vi "create available tags menu.vi"(5 "reference":refnum<vi>, 7 "channel action event":refnum<user-event>, 8 "error in":errorcluster, 9 "channel to map to":refnum<class "TBM channel.lvclass">, 10 "Coords":T1, 11 "engine configuration in":refnum<class "engine configuration.lvclass">) -> (0 "error out":errorcluster)   [LabVIEW 2013, in "control module editor.lvclass"]
uses:
  control module editor.lvclass
  <vilib>/NI/Module Execution Interface/Engine Configuration/engine configuration.lvclass
  <vilib>/NI/Tag Bus Module Framework/channel/TBM channel.lvclass
  Table API/Available Tag Menu/channel action event.ctl
  Table API/Available Tag Menu/dialog output action.ctl
  <vilib>/NI/Tag Bus/tag/tag descriptor.lvclass
  Table API/Table Manager/Call Back Ref Type Def.ctl
  Configuration Editor/Classes/Engine Parent/Engine Parent Editor Node.lvclass
  Configuration Editor/Classes/Module editor node/module editor node.lvclass
  <vilib>/Utility/miscctls.llb/LVPoint32TypeDef.ctl
  tag select dialog.vi
  Table API/Table Manager.lvlib
  Table API/Table Manager/Table Manager.lvclass
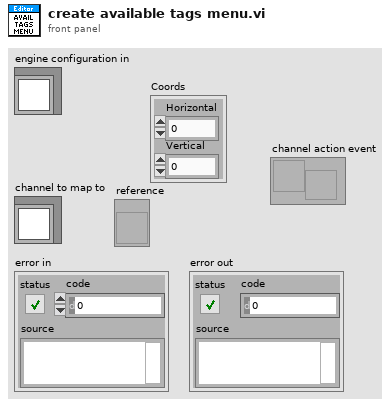
[diagram p1: front panel]
types:
  T1 = typedef "LVPoint32TypeDef.ctl" = cluster{"Horizontal":i32, "Vertical":i32}
  T2 = enum32{"Invalid", "Standard", "Closed", "Hidden", "Minimized", "Maximized"}
  T3 = typedef "LVRectTypeDef.ctl" = cluster{"Left":i16, "Top":i16, "Right":i16, "Bottom":i16}
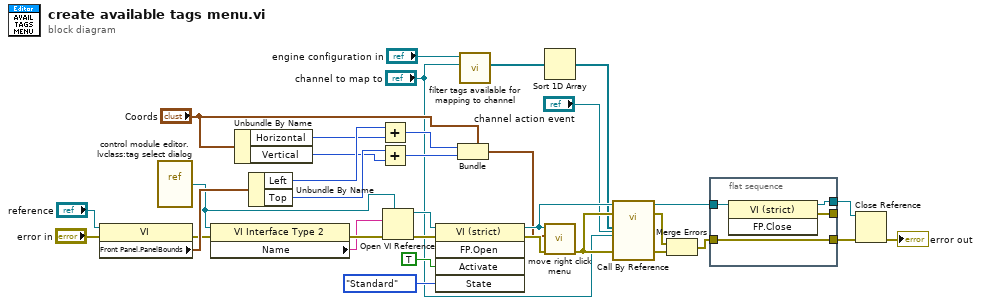
[diagram p0: block diagram]
diagram:
  n1 = property class="VI"(reference="reference", error in="error in") -> (error out=w9:errorcluster, "Front Panel.PanelBounds"=w32:T3)  [unwired: 1 out]
  n2 = vi-ref "control module editor.lvclass:tag select dialog.vi"() -> (w16:refnum<vi>)
  n3 = property class="VI Interface Type 2"(reference=w16, error in=w9) -> (error out=w23:errorcluster, "Name"=w22:string)  [unwired: 1 out]
  n4 = Unbundle By Name("Coords") -> ("Horizontal"=w30:i32, "Vertical"=w27:i32)
  n5 = Unbundle By Name(w32) -> ("Left"=w31:i16, "Top"=w28:i16)
  n6 = Add(x=w31, y=w30) -> (x+y=w29:i32)
  n7 = Add(x=w28, y=w27) -> (x+y=w26:i32)
  n8 = Open VI Reference(type specifier VI Refnum (for type only)=w16, vi path=w22, error in (no error)=w23) -> (vi reference=w20:refnum<vi>, error out=w21:errorcluster)  [unwired: 3 in]
  n9 = invoke class="VI (strict)" method="FP.Open"(reference=w20, error in=w21, "Activate"=TRUE ("Activate?"), "State"=T2."Standard") -> (reference out=w15:refnum<vi>, error out=w17:errorcluster)  [unwired: 1 in, 3 out]
  n10 = Bundle(cluster="Coords", "Horizontal"=w29, "Vertical"=w26) -> (w3:T1)
  n11 = call <vilib>:"filter tags available for mapping to channel.vi"("channel to map to"="channel to map to", "engine configuration in"="engine configuration in") -> ("filtered tags"=w33:refnum<class "tag descriptor.lvclass">[])  [unwired: 8 in, 1 out]
  n12 = Sort 1D Array(array=w33) -> (sorted array=w5:refnum<class "tag descriptor.lvclass">[])
  n13 = call "move right click menu.vi"("error in"=w17, "Point32"=w3, "VI"=w15) -> ("error out"=w7:errorcluster)  [unwired: 8 in]
  n14 = call-by-ref "?"(reference=w15, error in=w7, "channel action event"="channel action event", "error in"=w7, "channel to map to"="channel to map to", "filtered tags"=w5) -> (reference out=w13:refnum<vi>, error out=w14:errorcluster, 0:"error out"=w8:errorcluster)  [unwired: 7 in]
  n15 = Merge Errors(w14, w8) -> (w2:errorcluster)
  n16 = flat-sequence {
    tunnel: w13 -> [w38]
    tunnel: [w37] -> w12
    tunnel: [w36] -> _
    tunnel: w2 -> [w35]
    tunnel: [w35] -> w1
    frame #0 {
      n17 = invoke class="VI (strict)" method="FP.Close"(reference=w38) -> (reference out=w37:refnum<vi>, error out=w36:errorcluster)  [unwired: 2 in, 1 out]
    }
  }
  n18 = Close Reference(reference=w12, error in (no error)=w1) -> (error out=→"error out":errorcluster)
